vi "Init.vi"(6 "Column Descriptors":T11[](array[typedef]) {"MinWidth" min=2 step=1; "AutoSizeMode" items=["None"=1, "ColumnHeader"=2, "AllCellsExceptHeader"=4, "AllCells"=6, "DisplayedCellsExceptHeader"=8, "DisplayedCells"=10, "Fill"=16]; "FillWeight" min=1 max=100}, 7 "Right-Click Menu":T1[](array[typedef])=[{"Menu Name"="Add", "Menu Options"=enum."Always Show"}, {"Menu Name"="Remove", "Menu Options"=enum."Show When Used"}, {"Menu Name"="Edit", "Menu Options"=enum."Show When Used"}], 8 "error in (no error)":errorcluster, 9 "Node object refs":T3, 10 "Event References":T4, 11 "Multi Column Listbox in":refnum<class "Multi Column Listbox.lvclass">) -> (0 "error out":errorcluster, 2 "Table Events":T15, 3 "Multi Column Listbox out":refnum<class "Multi Column Listbox.lvclass">)   [LabVIEW 2014, in "Table Manager.lvlib" / "Multi Column Listbox.lvclass"]
doc: "This VIs creates the Column Objects that the table will use based on the configuration recived, and register the events the table will use. Also creates the evetns that will be used by the table"
uses:
  Multi Column Listbox.lvclass
  Table Manager/Table Events.ctl
  Table Manager/Menu Select.ctl
  Column/Column Descriptor.ctl
  Column/Column.lvclass
  Column/Column Type.ctl
  <vilib>/NI/Tag Bus/tag/Data Type.ctl
  Table Manager/Call Back Ref Type Def.ctl
  Configuration Editor/Classes/Engine Parent/Engine Parent Editor Node.lvclass
  Configuration Editor/Classes/Module editor node/module editor node.lvclass
  Table Manager/references.ctl
  <vilib>/NI/Configuration Framework/Node/StopEvent.ctl
  <vilib>/NI/Configuration Framework/Node/RefreshUIEvent.ctl
  <vilib>/NI/Configuration Framework/Node/CacheState.ctl
  <vilib>/NI/Configuration Framework/Node/NodeChangeEvent.ctl
  <vilib>/NI/Configuration Framework/Node/NodeRef.ctl
  <vilib>/NI/Configuration Framework/Node/NISE_CEF_Node.lvclass
  Available Tag Menu/channel action event.ctl
  Available Tag Menu/dialog output action.ctl
  <vilib>/NI/Tag Bus Module Framework/channel/TBM channel.lvclass
  <vilib>/NI/Tag Bus/tag/tag descriptor.lvclass
  <vilib>/NI/AMC/Message Queue.ctl
  <vilib>/NI/AMC/Message.ctl
  <vilib>/NI/Tools/Keyed Array/KeyedArray.ctl
  <vilib>/NI/Configuration Framework/Node/UserEventRef.ctl
  <vilib>/NI/Configuration Framework/Controls/EventCluster.ctl
  Table Manager/object ref.ctl
  Table Manager/Menu Definition.ctl
  Table Manager/Menu Options.ctl
  Line/Line.lvclass
  Multi Column Listbox.lvclass/Multi Column Listbox.ctl
  Table Manager/Table Manager.lvclass/Table Manager.ctl
  String Column/String Column.lvclass
  Column/Column.lvclass/Column.ctl
  Listbox Enum Column/List Box Enum Column.lvclass
  Listbox Enum Column/List Box Enum Column.lvclass/List Box Enum Column.ctl
  Mapping Column/Mapping Column.lvclass
  Mapping Column/Mapping Column.lvclass/Mapping Column.ctl
  Line/Line.lvclass/Line.ctl
  Column/Write Header.vi
  Column/Write Read Only.vi
  Column/Write Call Back VI.vi
  Listbox Enum Column/Write Enum Reference.vi
  Mapping Column/Write Channel suffix.vi
  Column/Write Dependencies List.vi
  Mapping Column/Write Data Type Dependecy.vi
  Mapping Column/Write Name Dependecy.vi
  Read Listbox.vi
  Table Manager/Write ATM.vi
  Line/Write Line UID.vi
  Line/Write Columns.vi
  Table Manager/Write object refs.vi
  Table Manager/Write Line.vi
  Table Manager/Write Menu Selection.vi
  Table Manager.lvlib
  Table Manager/Table Manager.lvclass
  <vilib>/NI/Tools/Keyed Array/Tools_KeyedArray.lvlib
  <vilib>/NI/AMC/AMC.lvlib
  <vilib>/NI/Configuration Framework/NISE_CEF_TreeControl.lvlib
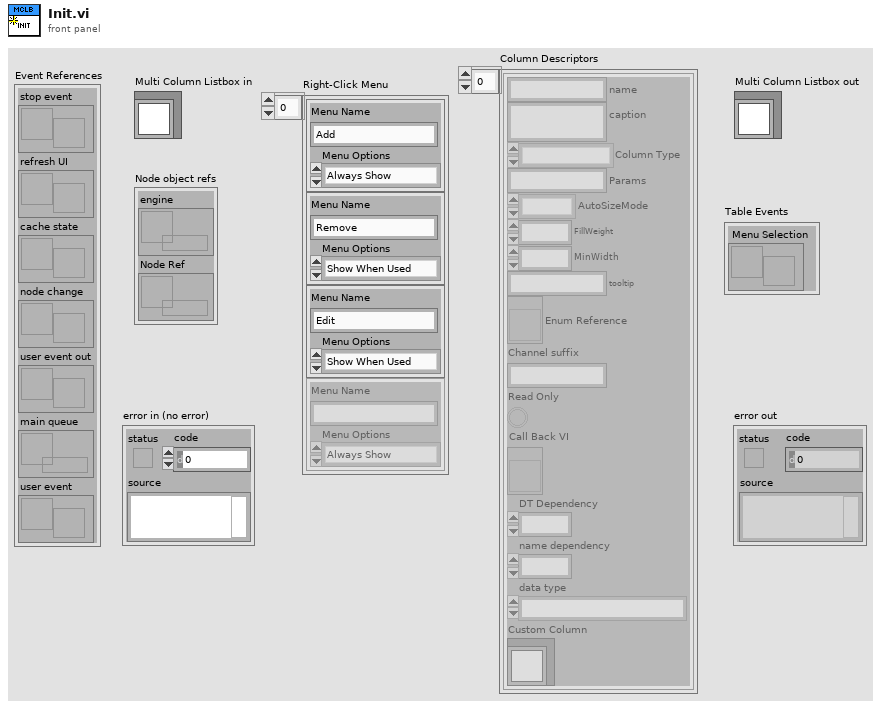
[diagram p1: front panel]
types:
  T1 = typedef "Table Manager.lvlib/Table Manager.lvclass/Menu Definition.ctl" = cluster{"Menu Name":string, "Menu Options":T2}
  T2 = typedef "Table Manager.lvlib/Table Manager.lvclass/Menu Options.ctl" = enum16{"Always Show", "Show When Used", "Show When Empty"}
  T3 = typedef "Table Manager.lvlib/Table Manager.lvclass/object ref.ctl" = cluster{"engine":refnum<data-value>, "Node Ref":refnum<data-value>}
  T4 = typedef "Table Manager.lvlib/Table Manager.lvclass/references.ctl" = cluster{"stop event":T5, "refresh UI":T6, "cache state":T7, "node change":T8, "user event out":refnum<user-event>, "main queue":T9, "user event":T10}
  T5 = typedef "NISE_CEF_Node.lvclass/StopEvent.ctl" = refnum<user-event>
  T6 = typedef "NISE_CEF_Node.lvclass/RefreshUIEvent.ctl" = refnum<user-event>
  T7 = typedef "NISE_CEF_Node.lvclass/CacheState.ctl" = refnum<user-event>
  T8 = typedef "NISE_CEF_Node.lvclass/NodeChangeEvent.ctl" = refnum<user-event>
  T9 = typedef "AMC.lvlib/Message Queue.ctl" = refnum<queue>
  T10 = typedef "NISE_CEF_Node.lvclass/UserEventRef.ctl" = refnum<user-event>
  T11 = typedef "Table Manager.lvlib/Column.lvclass/Column Descriptor.ctl" = cluster{"name":string, "caption":string, "Column Type":T12, "Params":string, "AutoSizeMode":i32, "FillWeight":sgl, "MinWidth":u32, "tooltip":string, "Enum Reference":refnum<vi>, "Channel suffix":string, "Read Only":bool, "Call Back VI":T13, "DT Dependency":i32, "name dependency":i32, "data type":T14, "Custom Column":refnum<class "Column.lvclass">}
  T12 = typedef "Table Manager.lvlib/Column.lvclass/Column Type.ctl" = enum16{"String", "Mapping", "Enum", "Custom"}
  T13 = typedef "Table Manager.lvlib/Table Manager.lvclass/Call Back Ref Type Def.ctl" = refnum<vi>
  T14 = typedef "tag bus.lvlib/tag descriptor.lvclass/Data Type.ctl" = enum16{"Double", "Single", "I64", "I32", "I16", "I8", "U64", "U32", "U16", "U8", "Boolean", "String", "Array of Double", "Array of Single", "Array of I64", "Array of I32", "Array of I16", "Array of I8", "Array of U64", "Array of U32", "Array of U16", "Array of U8", "Array of Boolean", "Array of String"}
  T15 = typedef "Table Manager.lvlib/Table Manager.lvclass/Table Events.ctl" = cluster{"Menu Selection":refnum<user-event>}
  T16 = typedef "Table Manager.lvlib/Table Manager.lvclass/Menu Select.ctl" = cluster{"Line Name":string, "Selected Value":string, "Row":i32, "Column":i32, "Table Index":i32}
  T17 = typedef "Table Manager.lvlib/channel action event.ctl" = cluster{"action":T18, "channel":refnum<class "TBM channel.lvclass">, "selected tag":refnum<class "tag descriptor.lvclass">, "Call Back VI":T13}
  T18 = typedef "Table Manager.lvlib/dialog output action.ctl" = enum16{"Tag Created", "Tag Selected", "Set Default", "disconnect"}
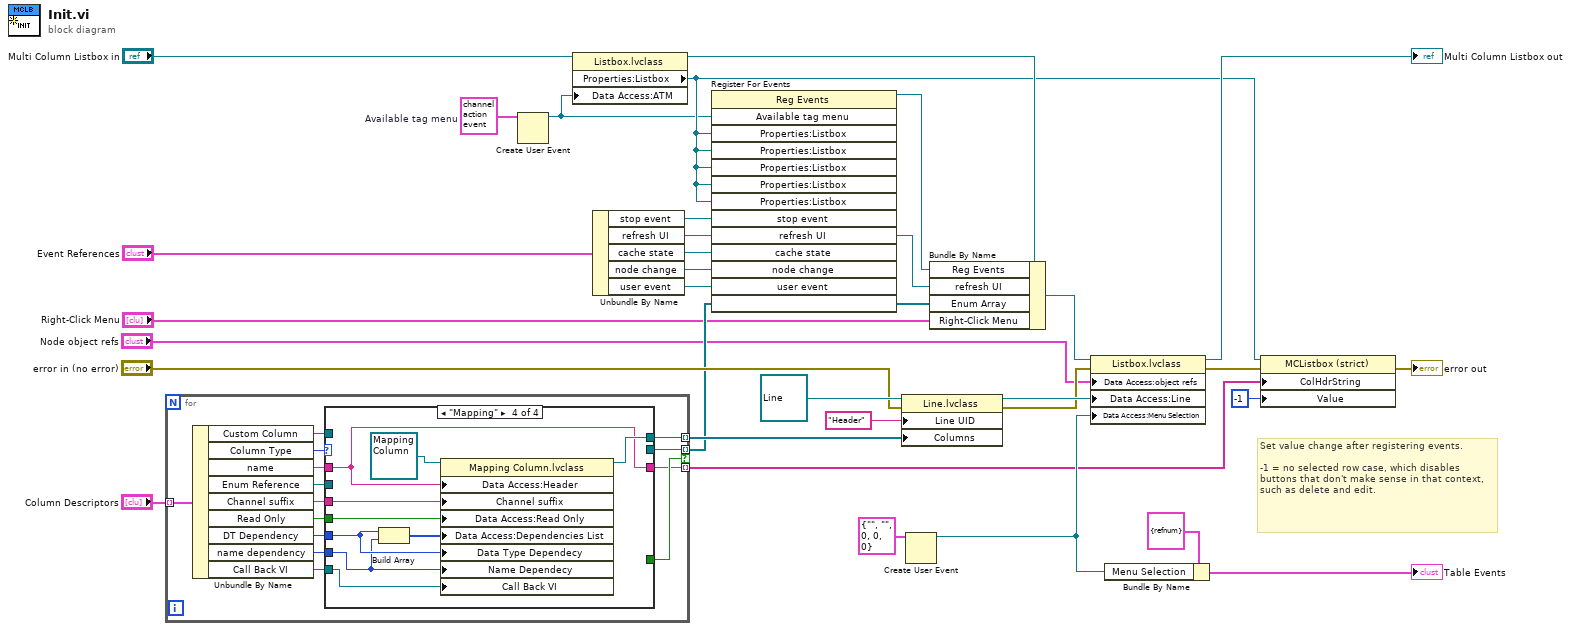
[diagram p0: block diagram]
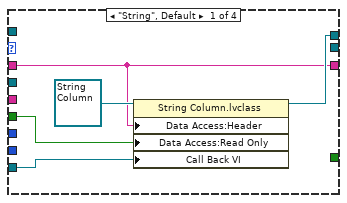
[diagram p2: hidden frame]
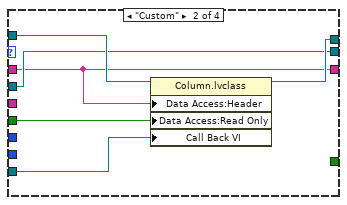
[diagram p3: hidden frame]
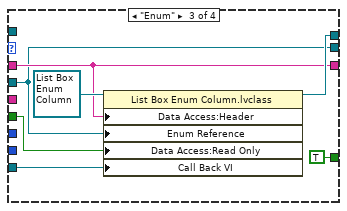
[diagram p4: hidden frame]
diagram:
  w24 = T17 {"action"=enum."Tag Created", "channel"=refnum, "selected tag"=refnum, "Call Back VI"=refnum}  # Available tag menu
  # "Set value change after registering events. \n\n-1 = no selected row case, which disables buttons that don't make sense in that context, such as delete and edit."
  n1 = for {
    tunnel: "Column Descriptors" -> [w46] mode=indexing
    tunnel: [w44] -> w29 mode=indexing
    tunnel: [w40] -> w17 mode=indexing if=w39
    tunnel: [w33] -> w9 mode=indexing
    n2 = Unbundle By Name(w46) -> ("Custom Column"=w34:refnum<class "Column.lvclass">, "Column Type"=w45:T12, "name"=w43:string, "Enum Reference"=w42:refnum<vi>, "Channel suffix"=w41:string, "Read Only"=w38:bool, "DT Dependency"=w37:i32, "name dependency"=w36:i32, "Call Back VI"=w35:T13)
    n3 = case shown="\"Mapping\"" w45 {
      tunnel: [w50 w57 w63 w72] -> w44
      tunnel: w43 -> [w47 w52 w59 w66]
      tunnel: w42 -> [_ w53 w58 _]
      tunnel: w41 -> [_ _ _ w71]
      tunnel: [_ w53 w58 _] -> w40
      tunnel: [_ _ TRUE _] -> w39
      tunnel: w38 -> [w49 w56 w61 w70]
      tunnel: w37 -> [_ _ _ w68]
      tunnel: w36 -> [_ _ _ w65]
      tunnel: w35 -> [w48 w55 w60 w67]
      tunnel: w34 -> [_ w54 _ _]
      tunnel: [w47 w52 w59 w66] -> w33
      frame "String", Default {
        n4 = property class="String Column.lvclass"(reference=refnum<class "String Column.lvclass"> refnum ("Table Manager.lvlib:String Column.lvclass"), "Data Access:Header"=w47, "Data Access:Read Only"=w49, "Call Back VI"=w48) -> (reference out=w50:refnum<class "String Column.lvclass">)  [unwired: 1 in, 1 out]
      }
      frame "Custom" {
        n5 = property class="Column.lvclass"(reference=w54, "Data Access:Header"=w52, "Data Access:Read Only"=w56, "Call Back VI"=w55) -> (reference out=w57:refnum<class "Column.lvclass">)  [unwired: 1 in, 1 out]
      }
      frame "Enum" {
        n6 = property class="List Box Enum Column.lvclass"(reference=refnum<class "List Box Enum Column.lvclass"> refnum ("Table Manager.lvlib:List Box Enum Column.lvclass"), "Data Access:Header"=w59, "Enum Reference"=w58, "Data Access:Read Only"=w61, "Call Back VI"=w60) -> (reference out=w63:refnum<class "List Box Enum Column.lvclass">)  [unwired: 1 in, 1 out]
      }
      frame "Mapping" {
        n7 = Build Array(w68, w65) -> (w69:i32[])
        n8 = property class="Mapping Column.lvclass"(reference=refnum<class "Mapping Column.lvclass"> refnum ("Table Manager.lvlib:Tag Channel Column.lvclass"), "Data Access:Header"=w66, "Channel suffix"=w71, "Data Access:Read Only"=w70, "Data Access:Dependencies List"=w69, "Data Type Dependecy"=w68, "Name Dependecy"=w65, "Call Back VI"=w67) -> (reference out=w72:refnum<class "Mapping Column.lvclass">)  [unwired: 1 in, 1 out]
      }
    }
  }
  n9 = Create User Event(user event datatype=w24) -> (user event=w2:refnum<user-event>)  [unwired: 1 in, 1 out]
  n10 = property class="Listbox.lvclass"(reference="Multi Column Listbox in", "Data Access:ATM"=w2) -> (reference out=w25:refnum<class "Multi Column Listbox.lvclass">, "Properties:Listbox"=w3:refnum<vi>)  [unwired: 1 in, 1 out]
  n11 = Unbundle By Name("Event References") -> ("stop event"=w22:T5, "refresh UI"=w4:T6, "cache state"=w21:T7, "node change"=w20:T8, "user event"=w19:T10)
  n12 = register-events(w2, w3, w3, w3, w3, w3, w22, w4, w21, w20, w19, w17) -> (reference out=w16:refnum<event-registration>)  [unwired: 2 in, 1 out]
  n13 = property class="Line.lvclass"(reference=refnum<class "Line.lvclass"> refnum ("Table Manager.lvlib:Line.lvclass"), error in="error in (no error)", "Line UID"="Header", "Columns"=w29) -> (reference out=w27:refnum<class "Line.lvclass">, error out=w11:errorcluster)
  n14 = Create User Event(user event datatype=T16 {"Line Name"="", "Selected Value"="", "Row"=0, "Column"=0, "Table Index"=0} ("Menu Selection")) -> (user event=w12:refnum<user-event>)  [unwired: 1 in, 1 out]
  n15 = Bundle By Name(cluster=w25, "Reg Events"=w16, "refresh UI"=w4, "Enum Array"=w17, "Right-Click Menu"="Right-Click Menu") -> (w5:refnum<class "Multi Column Listbox.lvclass">)
  n16 = property class="Listbox.lvclass"(reference=w5, error in=w11, "Data Access:object refs"="Node object refs", "Data Access:Line"=w27, "Data Access:Menu Selection"=w12) -> (reference out=→"Multi Column Listbox out":refnum<class "Multi Column Listbox.lvclass">, error out=w7:errorcluster)
  n17 = Bundle By Name(cluster=T15 {"Menu Selection"=refnum} ("Table Events"), "Menu Selection"=w12) -> (→"Table Events":T15)
  n18 = property class="MCListbox (strict)"(reference=w3, error in=w7, "ColHdrString"=w9, "Value"=-1) -> (error out=→"error out":errorcluster)  [unwired: 1 out]
